vi "JsonRpcRequestClusterToString.vi"(8 "error in (no error)":errorcluster, 10 "JsonRPCHttpRequestBody":T1) -> (0 "error out":errorcluster, 2 "JsonRpcHttpRequestBodyJsonString":string)   [LabVIEW 2017]
uses:
  <vilib>/LVH/i3 JSON/JSON Generation/Create Value Files/Create Value - Object.vi
  <vilib>/LVH/i3 JSON/JSON Generation/Add Object Parameter Files/Add Object Parameter - String.vi
  <vilib>/LVH/i3 JSON/JSON Generation/Add Object Parameter Files/Add Object Parameter - Object.vi
  <vilib>/LVH/i3 JSON/i3-json.lvlib
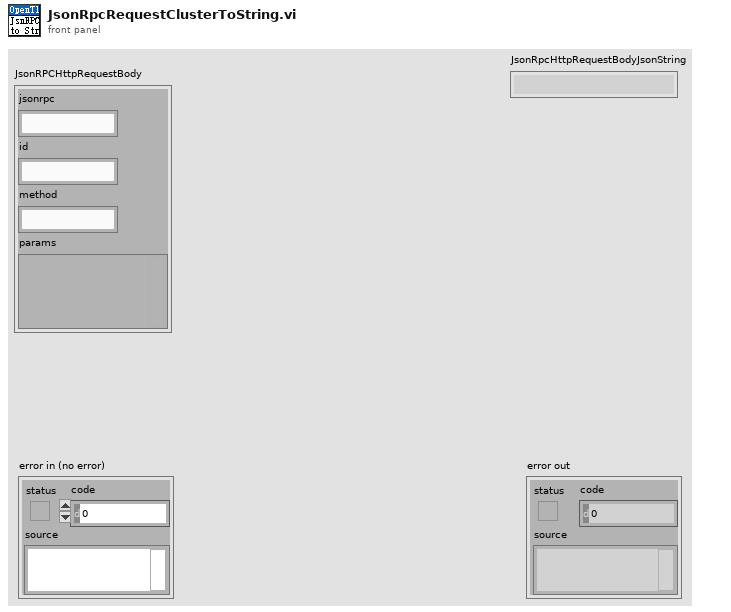
[diagram p1: front panel]
types:
  T1 = cluster{"jsonrpc":string, "id":string, "method":string, "params":variant}
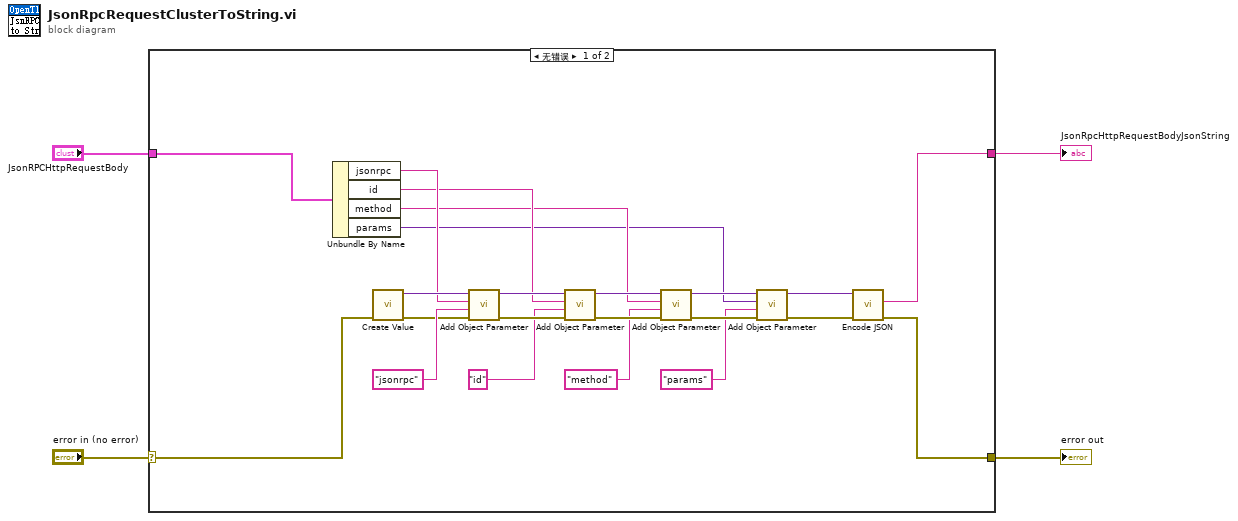
[diagram p0: block diagram]
diagram:
  n1 = case shown="无错误" "error in (no error)" {
    selector: "error in (no error)" -> [w5 w27]
    tunnel: [w7 w27] -> w3
    tunnel: "JsonRPCHttpRequestBody" -> [w26 _]
    tunnel: [w8 _] -> w1
    frame No Error {
      n2 = Unbundle By Name(w26) -> ("jsonrpc"=w23:string, "id"=w20:string, "method"=w16:string, "params"=w12:variant)
      n3 = call-poly <vilib>:"Create Value.vi"("error in (no error)"=w5) -> ("error out"=w6:errorcluster, "JSON Tree"=w25:variant)  [unwired: 9 in]
      n4 = call-poly <vilib>:"Add Object Parameter.vi"("error in (no error)"=w6, "Name"="jsonrpc", "String"=w23, "JSON Tree in (JSON Object)"=w25) -> ("error out"=w21:errorcluster, "JSON Tree out (JSON Object)"=w22:variant)  [unwired: 6 in]
      n5 = call-poly <vilib>:"Add Object Parameter.vi"("error in (no error)"=w21, "Name"="id", "String"=w20, "JSON Tree in (JSON Object)"=w22) -> ("error out"=w17:errorcluster, "JSON Tree out (JSON Object)"=w18:variant)  [unwired: 6 in]
      n6 = call-poly <vilib>:"Add Object Parameter.vi"("error in (no error)"=w17, "Name"="method", "String"=w16, "JSON Tree in (JSON Object)"=w18) -> ("error out"=w13:errorcluster, "JSON Tree out (JSON Object)"=w14:variant)  [unwired: 6 in]
      n7 = call-poly <vilib>:"Add Object Parameter.vi"("error in (no error)"=w13, "Name"="params", "JSON Object"=w12, "JSON Tree in (JSON Object)"=w14) -> ("error out"=w10:errorcluster, "JSON Tree out (JSON Object)"=w9:variant)  [unwired: 6 in]
      n8 = call <vilib>:"Encode JSON.vi"("error in (no error)"=w10, "JSON Tree"=w9) -> ("error out"=w7:errorcluster, "String"=w8:string)  [unwired: 4 in]
    }
    frame Error {
    }
  }
  "error out" <- w3
  "JsonRpcHttpRequestBodyJsonString" <- w1
